vi "Producer Consumer Main.vi"() -> ()   [LabVIEW 2021]
uses:
  Motor/Type_Defs/Control_Mode.ctl
  UI_Command.ctl
  Command.ctl
  Consumer State.ctl
  Motor/Motor.lvclass
  Elevator/Elevator.lvclass
  Modbus_Master/Modbus_Master.lvclass
  System_Telemetry.ctl
panel:
  out "Consumer Error Code":errorcluster
  out "Drive Diagnostics":T1
  out "Waveform Chart":T2(graph)
  in  "Stop Button":bool
  in  "Reset Fault":bool
  in  "Motor Control Mode":T3
  in  "Target Position":dbl
  in  "Target Torque":dbl
  in  "Target Speed":dbl
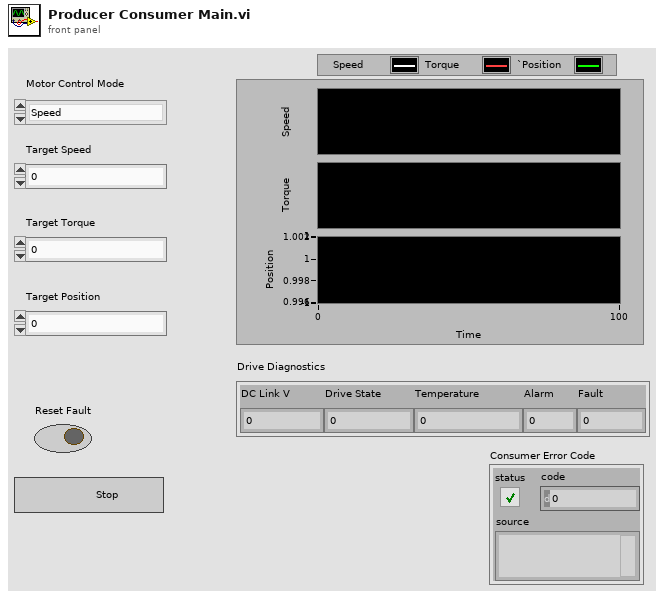
[diagram p1: front panel]
types:
  T1 = cluster{"DC Link V":dbl, "Drive State":u16, "Temperature":dbl, "Alarm":dbl, "Fault":dbl}
  T2 = cluster{"Actual Speed (RPM)":dbl, "Actual Torque (Nm)":dbl, "Actual Position (mm)":dbl}
  T3 = typedef "Motor.lvclass/Control_Mode.ctl" = enum16{"Speed", "Torque"}
  T4 = typedef "System_Telemetry.ctl" = cluster{"Actual Speed (RPM)":dbl, "Actual Torque (Nm)":dbl, "Actual Position (mm)":dbl, "Drive Diagnostics":cluster{"Fault":dbl, "Alarm":dbl, "Drive State":u16, "DC Link V":dbl, "Temperature":dbl}, "error in (no error)":errorcluster}
  T5 = typedef "Consumer State.ctl" = cluster{"Motor.lvclass":refnum<class "Motor.lvclass">, "Elevator.lvclass":refnum<class "Elevator.lvclass">, "Modbus_Master.lvclass":refnum<class "Modbus_Master.lvclass">, "Target Motor Cmd":dbl, "Target Position Cmd":dbl, "Loop Counter":i32}
  T6 = typedef "UI_Command.ctl" = cluster{"Command":T7, "Target RPM":dbl, "Target Torque":dbl, "Target Position":dbl, "Enable State":bool, "Motor Control Mode":T3}
  T7 = typedef "Command.ctl" = enum16{"Control & Read", "Enable Motor", "Set Motor Mode", "Set Motor Setpoint", "Set Elevator Setpoint", "Reset Fault", "Shutdown"}
  T8 = typedef "Device Context Cluster.ctl" = cluster{"Motor in":refnum<class "Motor.lvclass">, "Elevator.lvclass":refnum<class "Elevator.lvclass">, "Modbus_Master.lvclass":refnum<class "Modbus_Master.lvclass">, "ServoDrive.lvclass":refnum<class "ServoDrive.lvclass">}
  T9 = cluster{"DC Link V":dbl, "Drive State":u16, "Heatsink Temp C":dbl, "Alarm Code":dbl, "Fauld Code":dbl}
  T10 = cluster{"Fault":dbl, "Alarm":dbl, "Drive State":u16, "DC Link V":dbl, "Temperature":dbl}
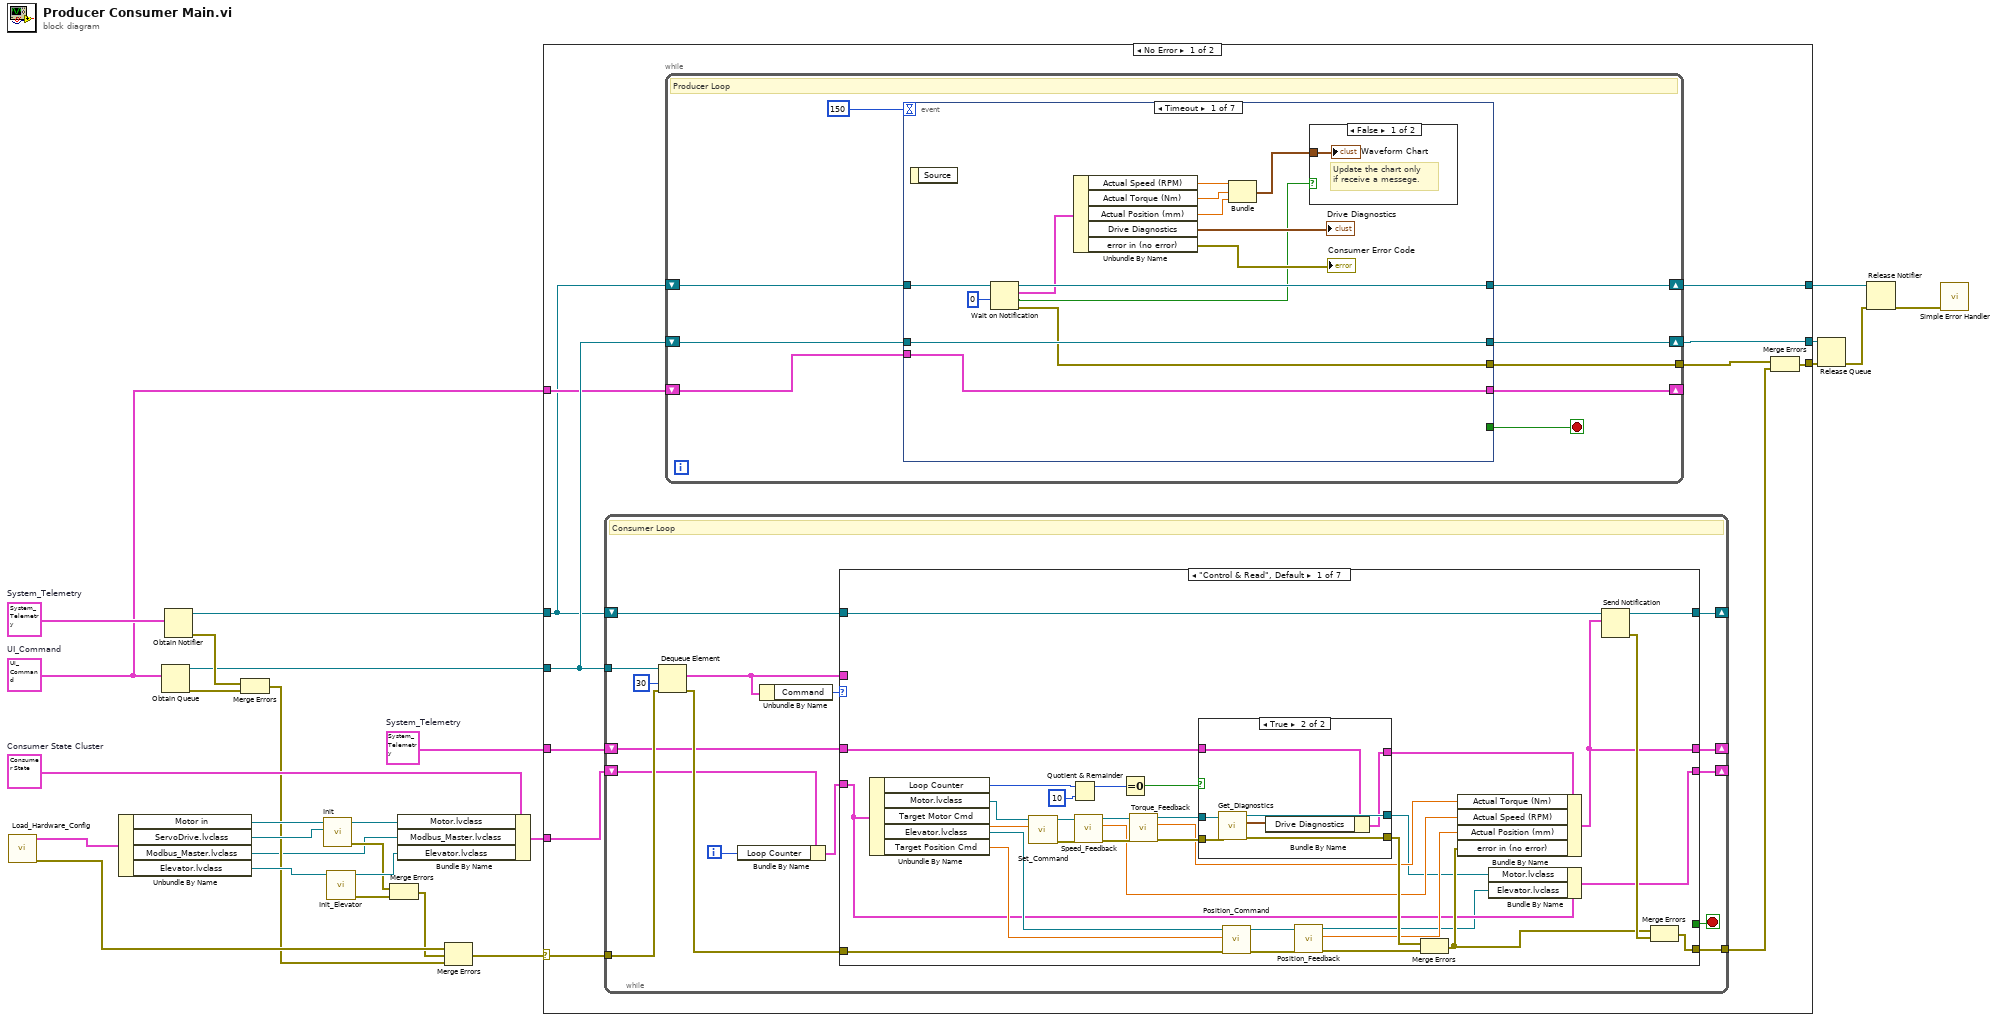
[diagram p0: block diagram]
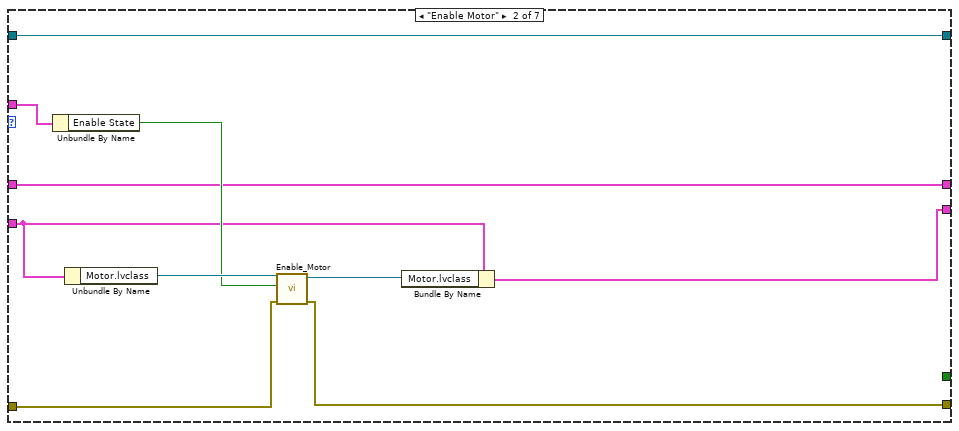
[diagram p3: hidden frame]
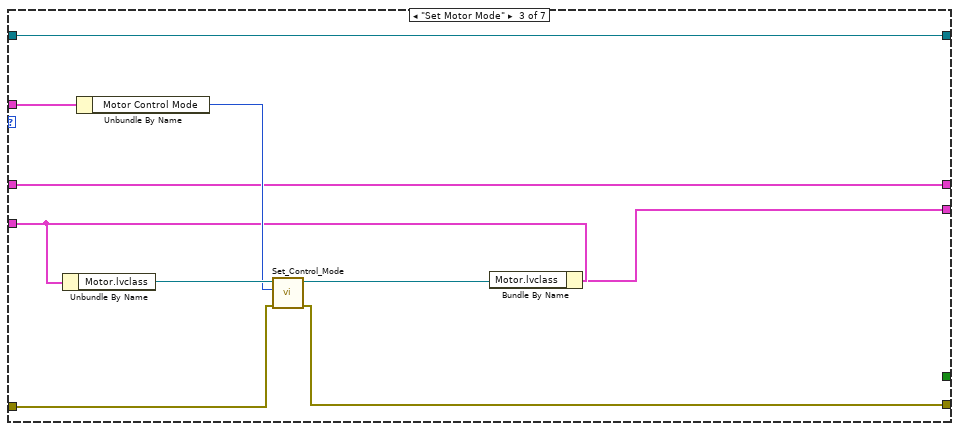
[diagram p4: hidden frame]
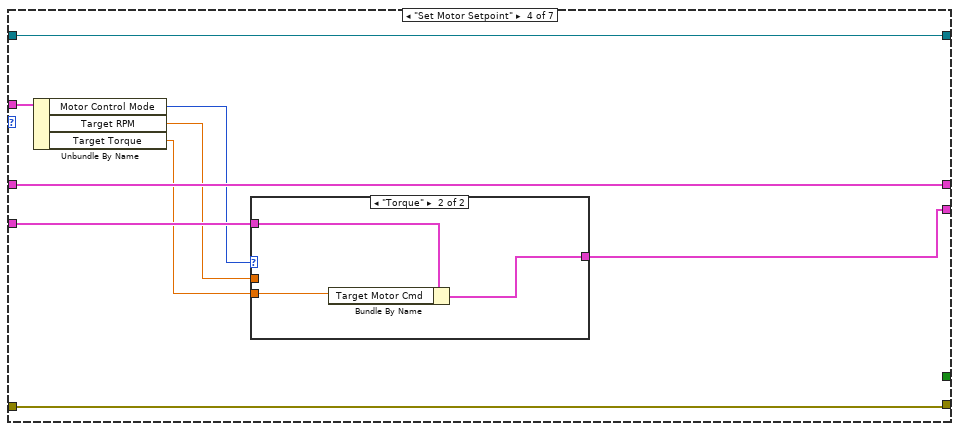
[diagram p5: hidden frame]
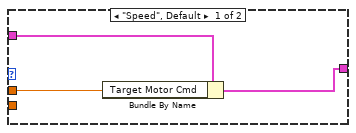
[diagram p6: hidden frame]
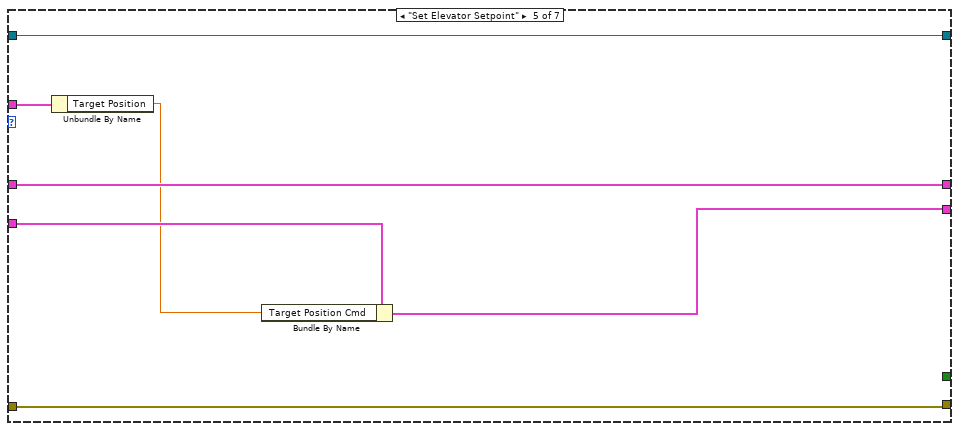
[diagram p7: hidden frame]
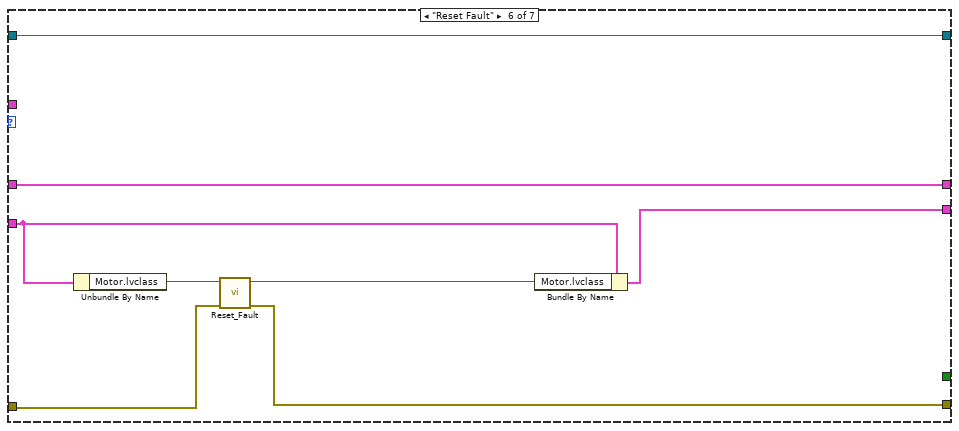
[diagram p8: hidden frame]
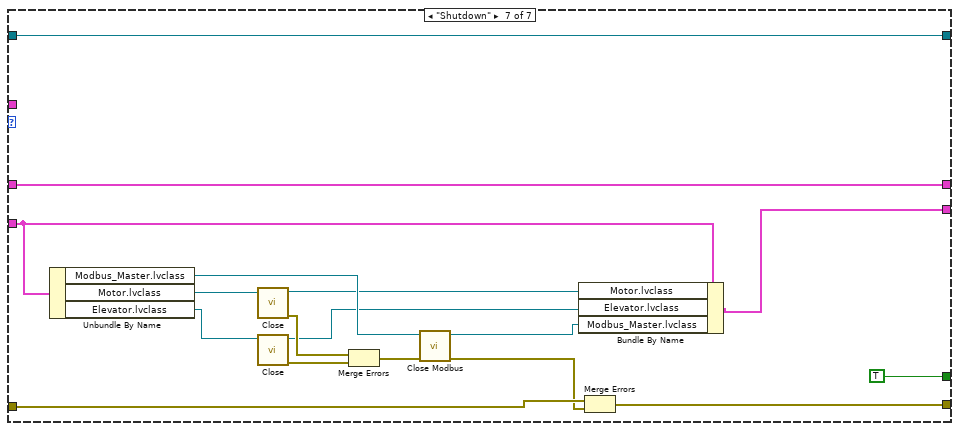
[diagram p9: hidden frame]
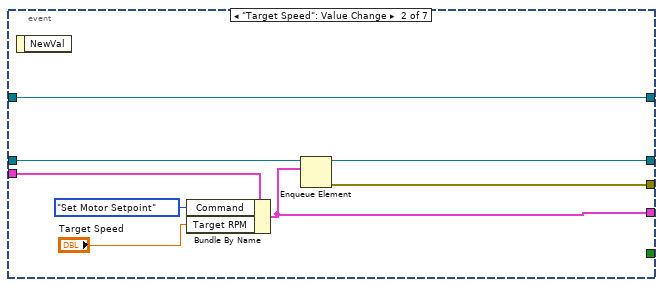
[diagram p11: hidden frame]
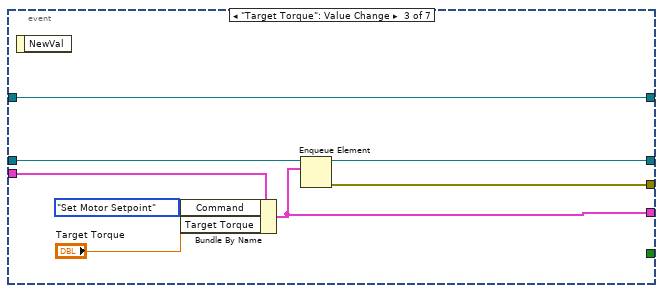
[diagram p12: hidden frame]
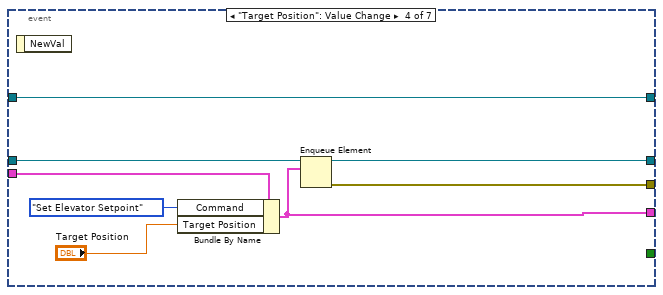
[diagram p13: hidden frame]
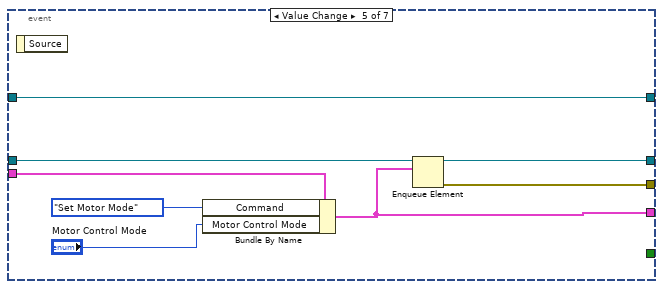
[diagram p14: hidden frame]
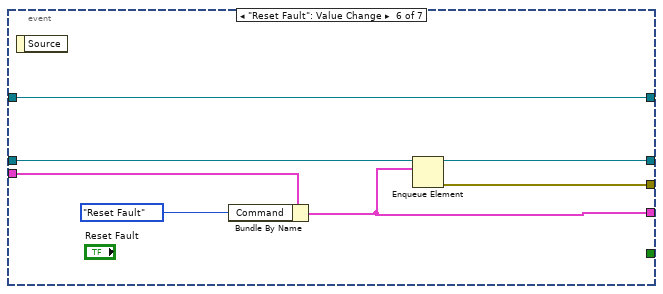
[diagram p15: hidden frame]
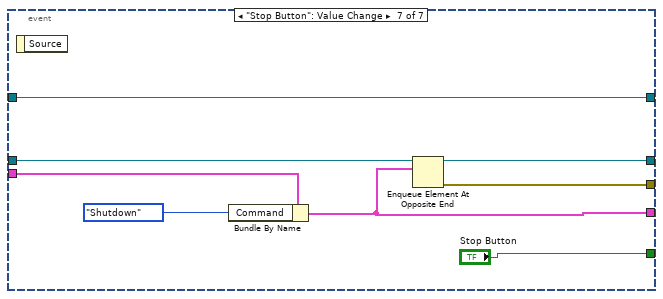
[diagram p16: hidden frame]
diagram:
  w22 = T4 {"Actual Speed (RPM)"=0.0, "Actual Torque (Nm)"=0.0, "Actual Position (mm)"=0.0, "Drive Diagnostics"={"Fault"=0.0, "Alarm"=0.0, "Drive State"=0, "DC Link V"=0.0, "Temperature"=0.0}, "error in (no error)"={"status"=FALSE, "code"=0, "source"=""}}  # System_Telemetry
  w21 = T5 {"Motor.lvclass"=refnum, "Elevator.lvclass"=refnum, "Modbus_Master.lvclass"=refnum, "Target Motor Cmd"=0.0, "Target Position Cmd"=0.0, "Loop Counter"=0}  # Consumer State Cluster
  w27 = T4 {"Actual Speed (RPM)"=0.0, "Actual Torque (Nm)"=0.0, "Actual Position (mm)"=0.0, "Drive Diagnostics"={"Fault"=0.0, "Alarm"=0.0, "Drive State"=0, "DC Link V"=0.0, "Temperature"=0.0}, "error in (no error)"={"status"=FALSE, "code"=0, "source"=""}}  # System_Telemetry
  w9 = T6 {"Command"=enum."Control & Read", "Target RPM"=0.0, "Target Torque"=0.0, "Target Position"=0.0, "Enable State"=FALSE, "Motor Control Mode"=enum."Speed"}  # UI_Command
  n1 = call "Load_Hardware_Config.vi"() -> ("error out"=w14:errorcluster, "Device Context Cluster"=w26:T8)  [unwired: 10 in]
  n2 = Unbundle By Name(w26) -> ("Motor in"=w25:refnum<class "Motor.lvclass">, "ServoDrive.lvclass"=w23:refnum<class "ServoDrive.lvclass">, "Modbus_Master.lvclass"=w2:refnum<class "Modbus_Master.lvclass">, "Elevator.lvclass"=w24:refnum<class "Elevator.lvclass">)
  n3 = Obtain Queue(element data type=w9) -> (queue out=w10:refnum<queue>, error out=w17:errorcluster)  [unwired: 4 in, 1 out]
  n4 = Obtain Notifier(notification data type=w27) -> (notifier out=w8:refnum<notifier>, error out=w11:errorcluster)  [unwired: 3 in, 1 out]
  n5 = Merge Errors(w11, w17) -> (w12:errorcluster)
  n6 = call "Init.vi"("ServoDrive.lvclass"=w23, "Motor in"=w25) -> ("error out"=w15:errorcluster, "Motor out"=w20:refnum<class "Motor.lvclass">)  [unwired: 8 in]
  n7 = call "Init_Elevator.vi"("Elevator in"=w24) -> ("error out"=w16:errorcluster, "Elevator out"=w18:refnum<class "Elevator.lvclass">)  [unwired: 9 in]
  n8 = Merge Errors(w15, w16) -> (w13:errorcluster)
  n9 = Bundle By Name(cluster=w21, "Motor.lvclass"=w20, "Modbus_Master.lvclass"=w2, "Elevator.lvclass"=w18) -> (w19:T5)
  n10 = Merge Errors(w14, w13, w12) -> (w1:errorcluster)
  n11 = case shown="No Error" w1 {
    selector: w1 -> [w28 w237]
    tunnel: w22 -> [w38 _]
    tunnel: w19 -> [w37 _]
    tunnel: w10 -> [w36 w238]
    tunnel: w9 -> [w35 _]
    tunnel: w8 -> [w34 w239]
    tunnel: [w33 w238] -> w7
    tunnel: [w32 w239] -> w6
    tunnel: [w30 w237] -> w4
    frame No Error {
      n12 = while {
        tunnel: w36 -> [w53]
        tunnel: w28 -> [w51]
        shift-right: [w45] -> _
        shift-left: w37 -> [w41]
        shift-right: [w47] -> _
        shift-left: w34 -> [w48]
        tunnel: [w46] -> w29
        shift-right: [w43] -> _
        shift-left: w38 -> [w42]
        i -> [w39]
        stop <- w44 stop-if-true
        # "Consumer Loop"
        n13 = Dequeue Element(queue=w53, timeout in ms (-1)=30, error in (no error)=w51) -> (element=w50:T6, error out=w49:errorcluster)  [unwired: 2 out]
        n14 = Bundle By Name(cluster=w41, "Loop Counter"=w39) -> (w40:T5)
        n15 = Unbundle By Name(w50) -> ("Command"=w52:T7)
        n16 = case shown="\"Control & Read\", Default" w52 {
          tunnel: w50 -> [_ w107 w117 w122 w135 _ _]
          tunnel: w40 -> [w58 w103 w113 w127 w140 w145 w155]
          tunnel: w49 -> [w68 w105 w115 w125 w138 w143 w163]
          tunnel: w48 -> [w72 w100 w110 w124 w137 w148 w165]
          tunnel: [w71 w100 w110 w124 w137 w148 w165] -> w47
          tunnel: [w69 w104 w114 w125 w138 w142 w156] -> w46
          tunnel: [w55 w101 w111 w126 w139 w144 w151] -> w45
          tunnel: [_ _ _ _ _ _ TRUE] -> w44
          tunnel: [w66 w99 w109 w123 w136 w141 w149] -> w43
          tunnel: w42 -> [w61 w99 w109 w123 w136 w141 w149]
          frame "Control & Read", Default {
            n17 = Unbundle By Name(w58) -> ("Loop Counter"=w64:i32, "Motor.lvclass"=w88:refnum<class "Motor.lvclass">, "Target Motor Cmd"=w87:dbl, "Elevator.lvclass"=w81:refnum<class "Elevator.lvclass">, "Target Position Cmd"=w82:dbl)
            n18 = call "Set_Command.vi"("Motor Control"=w87, "Motor in"=w88) -> ("error out"=w85:errorcluster, "Motor out"=w86:refnum<class "Motor.lvclass">)  [unwired: 8 in]
            n19 = Quotient & Remainder(x=w64, y=10) -> (x-y*floor(x/y)=w78:i32)  [unwired: 1 out]
            n20 = call "Speed_Feedback.vi"("error in (no error)"=w85, "Motor in"=w86) -> ("error out"=w83:errorcluster, "Actual Speed"=w60:dbl, "Motor out"=w84:refnum<class "Motor.lvclass">)  [unwired: 7 in]
            n21 = Equal To 0?(x=w78) -> (x = 0?=w63:bool)
            n22 = call "Torque_Feedback.vi"("error in (no error)"=w83, "Motor in"=w84) -> ("error out"=w75:errorcluster, "Actual Torque"=w59:dbl, "Motor out"=w76:refnum<class "Motor.lvclass">)  [unwired: 7 in]
            n23 = case shown="True" w63 {
              tunnel: w76 -> [w91 w98]
              tunnel: w75 -> [w90 w97]
              tunnel: [w90 w96] -> w73
              tunnel: [w91 w95] -> w56
              tunnel: w61 -> [w89 w94]
              tunnel: [w89 w93] -> w65
              frame False {
              }
              frame True {
                n24 = call "Get_Diagnostics.vi"("error in (no error)"=w97, "Motor in"=w98) -> ("error out"=w96:errorcluster, "Diagnostics"=w92:T9, "Motor out"=w95:refnum<class "Motor.lvclass">)  [unwired: 7 in]
                n25 = Bundle By Name(cluster=w94, "Drive Diagnostics"=w92) -> (w93:T4)
              }
            }
            n26 = call "Position_Command.vi"("error in (no error)"=w68, "Elevator Position Control"=w82, "Elevator in"=w81) -> ("error out"=w79:errorcluster, "Elevator out"=w80:refnum<class "Elevator.lvclass">)  [unwired: 7 in]
            n27 = call-dynamic "Position_Feedback.vi"("error in (no error)"=w79, "Elevator in"=w80) -> ("error out"=w74:errorcluster, "Actual Position"=w62:dbl, "Elevator out"=w57:refnum<class "Elevator.lvclass">)  [unwired: 7 in]
            n28 = Merge Errors(w73, w74) -> (w67:errorcluster)
            n29 = Bundle By Name(cluster=w65, "Actual Torque (Nm)"=w59, "Actual Speed (RPM)"=w60, "Actual Position (mm)"=w62, "error in (no error)"=w67) -> (w66:T4)
            n30 = Bundle By Name(cluster=w58, "Motor.lvclass"=w56, "Elevator.lvclass"=w57) -> (w55:T5)
            n31 = Send Notification(notification=w66, notifier=w72) -> (notifier out=w71:refnum<notifier>, error out=w70:errorcluster)  [unwired: 1 in]
            n32 = Merge Errors(w67, w70) -> (w69:errorcluster)
          }
          frame "Enable Motor" {
            n33 = Unbundle By Name(w107) -> ("Enable State"=w106:bool)
            n34 = Unbundle By Name(w103) -> ("Motor.lvclass"=w108:refnum<class "Motor.lvclass">)
            n35 = call "Enable_Motor.vi"("error in (no error)"=w105, "Enable Drive"=w106, "Motor in"=w108) -> ("error out"=w104:errorcluster, "Motor out"=w102:refnum<class "Motor.lvclass">)  [unwired: 7 in]
            n36 = Bundle By Name(cluster=w103, "Motor.lvclass"=w102) -> (w101:T5)
          }
          frame "Set Motor Mode" {
            n37 = Unbundle By Name(w113) -> ("Motor.lvclass"=w118:refnum<class "Motor.lvclass">)
            n38 = Unbundle By Name(w117) -> ("Motor Control Mode"=w116:T3)
            n39 = call "Set_Control_Mode.vi"("error in (no error)"=w115, "Control Mode"=w116, "Motor in"=w118) -> ("error out"=w114:errorcluster, "Motor out"=w112:refnum<class "Motor.lvclass">)  [unwired: 7 in]
            n40 = Bundle By Name(cluster=w113, "Motor.lvclass"=w112) -> (w111:T5)
          }
          frame "Set Motor Setpoint" {
            n41 = Unbundle By Name(w122) -> ("Motor Control Mode"=w121:T3, "Target RPM"=w119:dbl, "Target Torque"=w120:dbl)
            n42 = case shown="\"Torque\"" w121 {
              tunnel: w127 -> [w130 w133]
              tunnel: [w128 w132] -> w126
              tunnel: w120 -> [_ w131]
              tunnel: w119 -> [w129 _]
              frame "Speed", Default {
                n43 = Bundle By Name(cluster=w130, "Target Motor Cmd"=w129) -> (w128:T5)
              }
              frame "Torque" {
                n44 = Bundle By Name(cluster=w133, "Target Motor Cmd"=w131) -> (w132:T5)
              }
            }
          }
          frame "Set Elevator Setpoint" {
            n45 = Unbundle By Name(w135) -> ("Target Position"=w134:dbl)
            n46 = Bundle By Name(cluster=w140, "Target Position Cmd"=w134) -> (w139:T5)
          }
          frame "Reset Fault" {
            n47 = Unbundle By Name(w145) -> ("Motor.lvclass"=w147:refnum<class "Motor.lvclass">)
            n48 = call "Reset_Fault.vi"("error in (no error)"=w143, "Motor in"=w147) -> ("error out"=w142:errorcluster, "Motor out"=w146:refnum<class "Motor.lvclass">)  [unwired: 8 in]
            n49 = Bundle By Name(cluster=w145, "Motor.lvclass"=w146) -> (w144:T5)
          }
          frame "Shutdown" {
            n50 = Unbundle By Name(w155) -> ("Modbus_Master.lvclass"=w158:refnum<class "Modbus_Master.lvclass">, "Motor.lvclass"=w162:refnum<class "Motor.lvclass">, "Elevator.lvclass"=w164:refnum<class "Elevator.lvclass">)
            n51 = call "Close.vi"("Motor in"=w162) -> ("error out"=w160:errorcluster, "Motor out"=w154:refnum<class "Motor.lvclass">)  [unwired: 9 in]
            n52 = call-dynamic "Close.vi"("Elevator in"=w164) -> ("error out"=w161:errorcluster, "Elevator out"=w153:refnum<class "Elevator.lvclass">)  [unwired: 9 in]
            n53 = Merge Errors(w160, w161) -> (w159:errorcluster)
            n54 = call "Close Modbus.vi"("error in (no error)"=w159, "Modbus_Master in"=w158) -> ("error out"=w157:errorcluster, "Modbus_Master out"=w152:refnum<class "Modbus_Master.lvclass">)  [unwired: 8 in]
            n55 = Bundle By Name(cluster=w155, "Motor.lvclass"=w154, "Elevator.lvclass"=w153, "Modbus_Master.lvclass"=w152) -> (w151:T5)
            n56 = Merge Errors(w163, w157) -> (w156:errorcluster)
          }
        }
      }
      n57 = while {
        shift-right: [w172] -> _
        shift-left: w35 -> [w171]
        tunnel: [w170] -> w31
        shift-right: [w169] -> w33
        shift-left: w36 -> [w173]
        shift-right: [w167] -> w32
        shift-left: w34 -> [w168]
        stop <- w166 stop-if-true
        # "Producer Loop"
        n58 = event shown="[0] Timeout" {
          selector: _ -> [_ _ _ _ _ _ _]
          dyn-events: _ -> [_ _ _ _ _ _ _]
          timeout: 150 -> [_ _ _ _ _ _ _]
          tunnel: w173 -> [w188 w197 w205 w213 w221 w228 w236]
          tunnel: [w187 w194 w203 w211 w219 w226 w234] -> w172
          tunnel: w171 -> [w187 w193 w202 w210 w218 w225 w233]
          tunnel: [w185 w192 w201 w209 w217 w224 w232] -> w170
          tunnel: [w188 w191 w199 w208 w216 w223 w231] -> w169
          tunnel: w168 -> [w186 w190 w198 w206 w214 w222 w229]
          tunnel: [w184 w190 w198 w206 w214 w222 w229] -> w167
          tunnel: [_ _ _ _ _ _ "Stop Button"] -> w166
          event Timeout {
            n59 = event-data() -> ()  [unwired: 1 in, 1 out]
            n60 = Wait on Notification(notifier=w186, timeout in ms (-1)=0) -> (notifier out=w184:refnum<notifier>, notification=w183:T4, timed out?=w175:bool, error out=w185:errorcluster)  [unwired: 2 in]
            n61 = Unbundle By Name(w183) -> ("Actual Speed (RPM)"=w182:dbl, "Actual Torque (Nm)"=w181:dbl, "Actual Position (mm)"=w180:dbl, "Drive Diagnostics"=→"Drive Diagnostics":T10, "error in (no error)"=→"Consumer Error Code":errorcluster)
            n62 = Bundle("Actual Speed (RPM)"=w182, "Actual Torque (Nm)"=w181, "Actual Position (mm)"=w180) -> (w179:T2)  [unwired: 1 in]
            n63 = case shown="False" w175 {
              tunnel: w179 -> [w189 _]
              frame False {
                # "Update the chart only\nif receive a messege."
                "Waveform Chart" <- w189
              }
              frame True {
              }
            }
          }
          event "Target Speed": Value Change {
            n64 = event-data() -> ()  [unwired: 1 in, 1 out]
            n65 = Bundle By Name(cluster=w193, "Command"=Command."Set Motor Setpoint", "Target RPM"="Target Speed") -> (w194:T6)
            n66 = Enqueue Element(queue=w197, element=w194) -> (queue out=w191:refnum<queue>, error out=w192:errorcluster)  [unwired: 2 in, 1 out]
          }
          event "Target Torque": Value Change {
            n67 = event-data() -> ()  [unwired: 1 in, 1 out]
            n68 = Bundle By Name(cluster=w202, "Command"=Command."Set Motor Setpoint", "Target Torque"="Target Torque") -> (w203:T6)
            n69 = Enqueue Element(queue=w205, element=w203) -> (queue out=w199:refnum<queue>, error out=w201:errorcluster)  [unwired: 2 in, 1 out]
          }
          event "Target Position": Value Change {
            n70 = event-data() -> ()  [unwired: 1 in, 1 out]
            n71 = Bundle By Name(cluster=w210, "Command"=Command."Set Elevator Setpoint", "Target Position"="Target Position") -> (w211:T6)
            n72 = Enqueue Element(queue=w213, element=w211) -> (queue out=w208:refnum<queue>, error out=w209:errorcluster)  [unwired: 2 in, 1 out]
          }
          event Value Change {
            n73 = event-data() -> ()  [unwired: 1 in, 1 out]
            n74 = Bundle By Name(cluster=w218, "Command"=Command."Set Motor Mode", "Motor Control Mode"="Motor Control Mode") -> (w219:T6)
            n75 = Enqueue Element(queue=w221, element=w219) -> (queue out=w216:refnum<queue>, error out=w217:errorcluster)  [unwired: 2 in, 1 out]
          }
          event "Reset Fault": Value Change {
            n76 = event-data() -> ()  [unwired: 1 in, 1 out]
            n77 = Bundle By Name(cluster=w225, "Command"=Command."Reset Fault") -> (w226:T6)
            n78 = Enqueue Element(queue=w228, element=w226) -> (queue out=w223:refnum<queue>, error out=w224:errorcluster)  [unwired: 2 in, 1 out]
          }
          event "Stop Button": Value Change {
            n79 = event-data() -> ()  [unwired: 1 in, 1 out]
            n80 = Bundle By Name(cluster=w233, "Command"=Command."Shutdown") -> (w234:T6)
            n81 = Enqueue Element At Opposite End(queue=w236, element=w234) -> (queue out=w231:refnum<queue>, error out=w232:errorcluster)  [unwired: 2 in, 1 out]
          }
        }
      }
      n82 = Merge Errors(w31, w29) -> (w30:errorcluster)
    }
    frame Error {
    }
  }
  n83 = Release Queue(queue=w7, error in (no error)=w4) -> (error out=w5:errorcluster)  [unwired: 1 in, 2 out]
  n84 = Release Notifier(notifier=w6, error in (no error)=w5) -> (error out=w3:errorcluster)  [unwired: 1 in, 2 out]
  n85 = call <vilib>:"Simple Error Handler.vi"("error in (no error)"=w3) -> ()  [unwired: 4 in, 5 out]
